vi "GOOP_DrawProductPicture.vi"(10 "BAckground ColorPane Color":u32(colorbox)=16777216, 11 "ProductPictureControl":refnum<vi>) -> (3 "Zoom Factor":sgl)   [LabVIEW 2020]
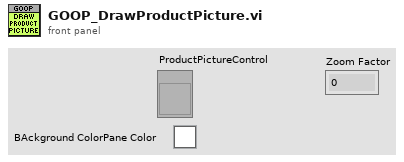
[diagram p1: front panel]
types:
  T1 = typedef "LVBoundsTypeDef.ctl" = cluster{"Width":u32, "Height":u32}
  T2 = typedef "imagedata.ctl" = cluster{"image type":i32, "image depth":i32, "image":u8[], "mask":u8[], "colors":u32[], "Rectangle":cluster{"left":i16, "top":i16, "right":i16, "bottom":i16}}
  T3 = cluster{"left":i16, "top":i16, "right":i16, "bottom":i16}
  T4 = cluster{"Width":u32, "Width":u32, "Width":u32, "Height":u32}
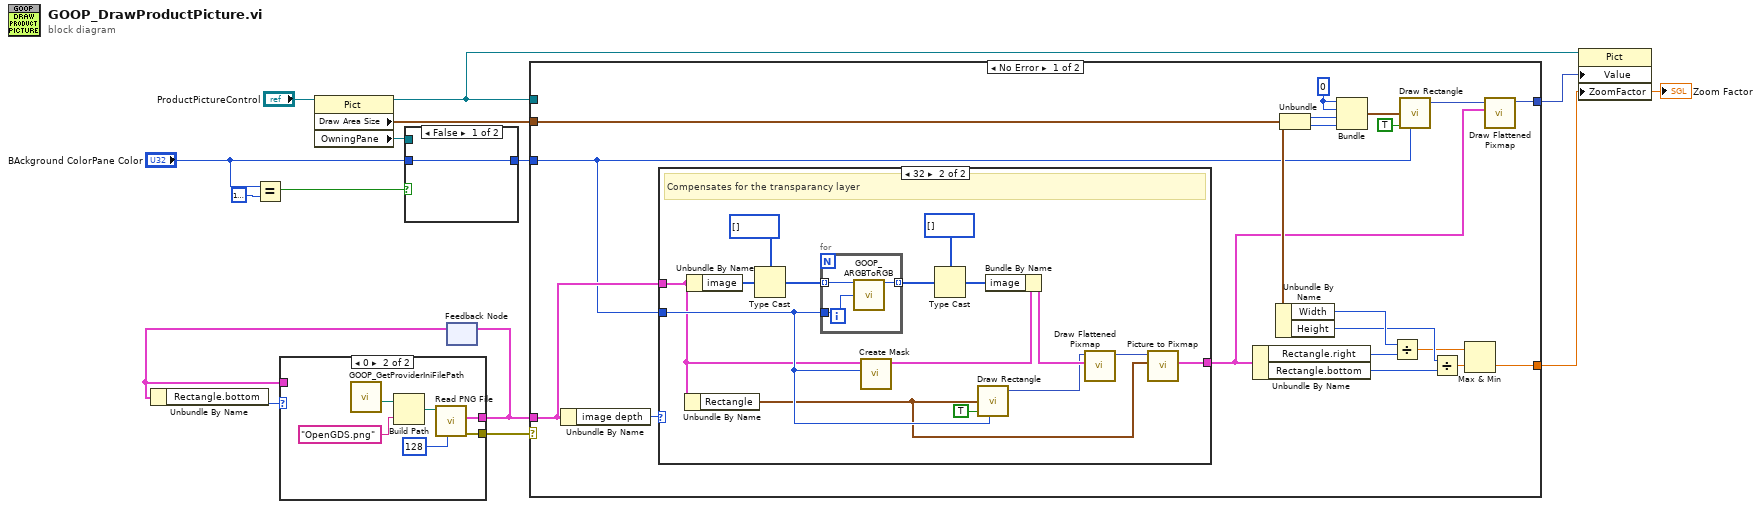
[diagram p0: block diagram]
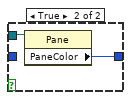
[diagram p2: hidden frame]
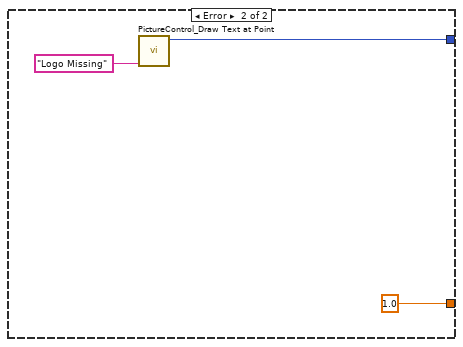
[diagram p4: hidden frame]
diagram:
  n1 = Equal?(x="BAckground ColorPane Color", y=u32 16777216) -> (x = y?=w2:bool)
  n2 = property class="Pict"(reference="ProductPictureControl") -> (reference out=w7:refnum<vi>, "Draw Area Size"=w5:T1, "OwningPane"=w6:refnum<vi>)  [unwired: 1 in, 1 out]
  n3 = case shown="False" w2 {
    tunnel: w6 -> [_ w17]
    tunnel: [w15 w16] -> w4
    tunnel: "BAckground ColorPane Color" -> [w15 _]
    frame False {
    }
    frame True {
      n4 = property class="Pane"(reference=w17) -> ("PaneColor"=w16:u32)  [unwired: 1 in, 2 out]
    }
  }
  n5 = feedback #1() -> (w14:T2)  [unwired: 1 in]
  n6 = Unbundle By Name(w14) -> ("Rectangle.bottom"=w9:i16)
  n7 = case shown="0" w9 {
    tunnel: [w18 w24] -> w10
    tunnel: w14 -> [w18 _]
    tunnel: [_ w20] -> w13
    frame Default {
    }
    frame 0 {
      n8 = call <resource>:"GOOP_GetProviderIniFilePath.vi"() -> ("ProviderMainFolder"=w23:path)  [unwired: 10 in, 1 out]
      n9 = Build Path(base path=w23, name or relative path="OpenGDS.png") -> (appended path=w21:path)
      n10 = call <vilib>:"Read PNG File.vi"("Transparency Thresh"=u8 128, "path to PNG file"=w21) -> ("error out"=w20:errorcluster, "image data"=w24:T2)  [unwired: 7 in, 1 out]
    }
  }
  n11 = feedback-in #1(w10) -> ()
  n12 = case shown="No Error" w13 {
    tunnel: w10 -> [w41 _]
    tunnel: [w43 w65] -> w12
    tunnel: [w27 sgl 1.0 ("Zoom Factor")] -> w11
    tunnel: w7 -> [_ _]
    tunnel: w5 -> [w29 _]
    tunnel: w4 -> [w28 _]
    frame No Error {
      w37 = u32 0 ("Width")
      n13 = Unbundle By Name(w41) -> ("image depth"=w42:i32)
      n14 = case shown="32" w42 {
        tunnel: w28 -> [_ w50]
        tunnel: w41 -> [w44 w49]
        tunnel: [w44 w45] -> w25
        frame Default {
        }
        frame 32 {
          # "Compensates for the transparancy layer"
          n15 = Unbundle By Name(w49) -> ("Rectangle"=w46:T3)
          n16 = Unbundle By Name(w49) -> ("image"=w58:u8[])
          n17 = Type Cast(type=u32[] [], x=w58) -> (*(type *) &x=w57:u32[])
          n18 = for {
            tunnel: w57 -> [w62] mode=indexing
            tunnel: w50 -> [w61]
            tunnel: [w60] -> w55 mode=indexing
            n19 = call <resource>:"GOOP_ARGBToRGB.vi"("ARGB"=w62, "BackgroundColor"=w61) -> ("RGB"=w60:u32)  [unwired: 12 in, 1 out]
          }
          n20 = call <vilib>:"Create Mask.vi"("Mask Color (Black)"=w50, "image data"=w49) -> ("image data"=w52:T2)  [unwired: 9 in]
          n21 = Type Cast(type=u8[] [] ("image"), x=w55) -> (*(type *) &x=w53:u8[])
          n22 = call <vilib>:"Draw Rectangle.vi"("rect"=w46, "fill?(F)"=TRUE, "color(black)"=w50) -> ("new picture"=w48:picture)  [unwired: 6 in]
          n23 = Bundle By Name(cluster=w52, "image"=w53) -> (w56:T2)
          n24 = call <vilib>:"Draw Flattened Pixmap.vi"("image data"=w56, "picture"=w48) -> ("new picture"=w47:picture)  [unwired: 7 in]
          n25 = call <vilib>:"Picture to Pixmap.vi"("rect"=w46, "picture"=w47) -> ("image data"=w45:T2)  [unwired: 8 in, 1 out]
        }
      }
      n26 = Unbundle By Name(w25) -> ("Rectangle.right"=w32:i16, "Rectangle.bottom"=w33:i16)
      n27 = Unbundle By Name(w29) -> ("Width"=w35:u32, "Height"=w34:u32)
      n28 = Unbundle(w29) -> ("Width"=w39:u32, "Height"=w38:u32)
      n29 = Bundle("Width"=w37, "Width"=w37, "Width"=w39, "Height"=w38) -> (w40:T4)  [unwired: 1 in]
      n30 = Divide(x=w35, y=w32) -> (x/y=w31:dbl)
      n31 = call <vilib>:"Draw Rectangle.vi"("rect"=w40, "fill?(F)"=TRUE, "color(black)"=w28) -> ("new picture"=w26:picture)  [unwired: 6 in]
      n32 = Divide(x=w34, y=w33) -> (x/y=w30:dbl)
      n33 = Max & Min(x=w31, y=w30) -> (min(x,y)=w27:dbl)  [unwired: 1 out]
      n34 = call <vilib>:"Draw Flattened Pixmap.vi"("image data"=w25, "picture"=w26) -> ("new picture"=w43:picture)  [unwired: 7 in]
    }
    frame Error {
      n35 = call <resource>:"PictureControl_Draw Text at Point.vi"("text"="Logo Missing") -> ("new picture"=w65:picture)  [unwired: 9 in, 1 out]
    }
  }
  "Zoom Factor" <- w11
  n36 = property class="Pict"(reference=w7, "Value"=w12, "ZoomFactor"=w11) -> ()  [unwired: 1 in, 2 out]
